vi "HEX-String Languages to Unicode Array.vi"(11 "Config in":T1) -> (3 "Config out":T1)   [LabVIEW 2019, in "Language Selection.lvlib"]
doc: "- - -\nCopyright (c) 2026, Merecs Engineering GmbH"
uses:
  Language Selection.lvlib
  TypeDefs/Cluster Language Configuration.ctl
  Cluster Settings Data.ctl
  TypeDefs/Cluster Language.ctl
  TypeDefs/Cluster PropertyTranslation.ctl
  TypeDefs/Enum Property Type.ctl
  <vilib>/addons/Tools/Unicode/_subVIs/Convert UTF-16LE to ASCII (Scalar).vi
  <vilib>/addons/Tools/Unicode/UI Unicode Tools.lvlib
panel:
  # "Connector Pane"
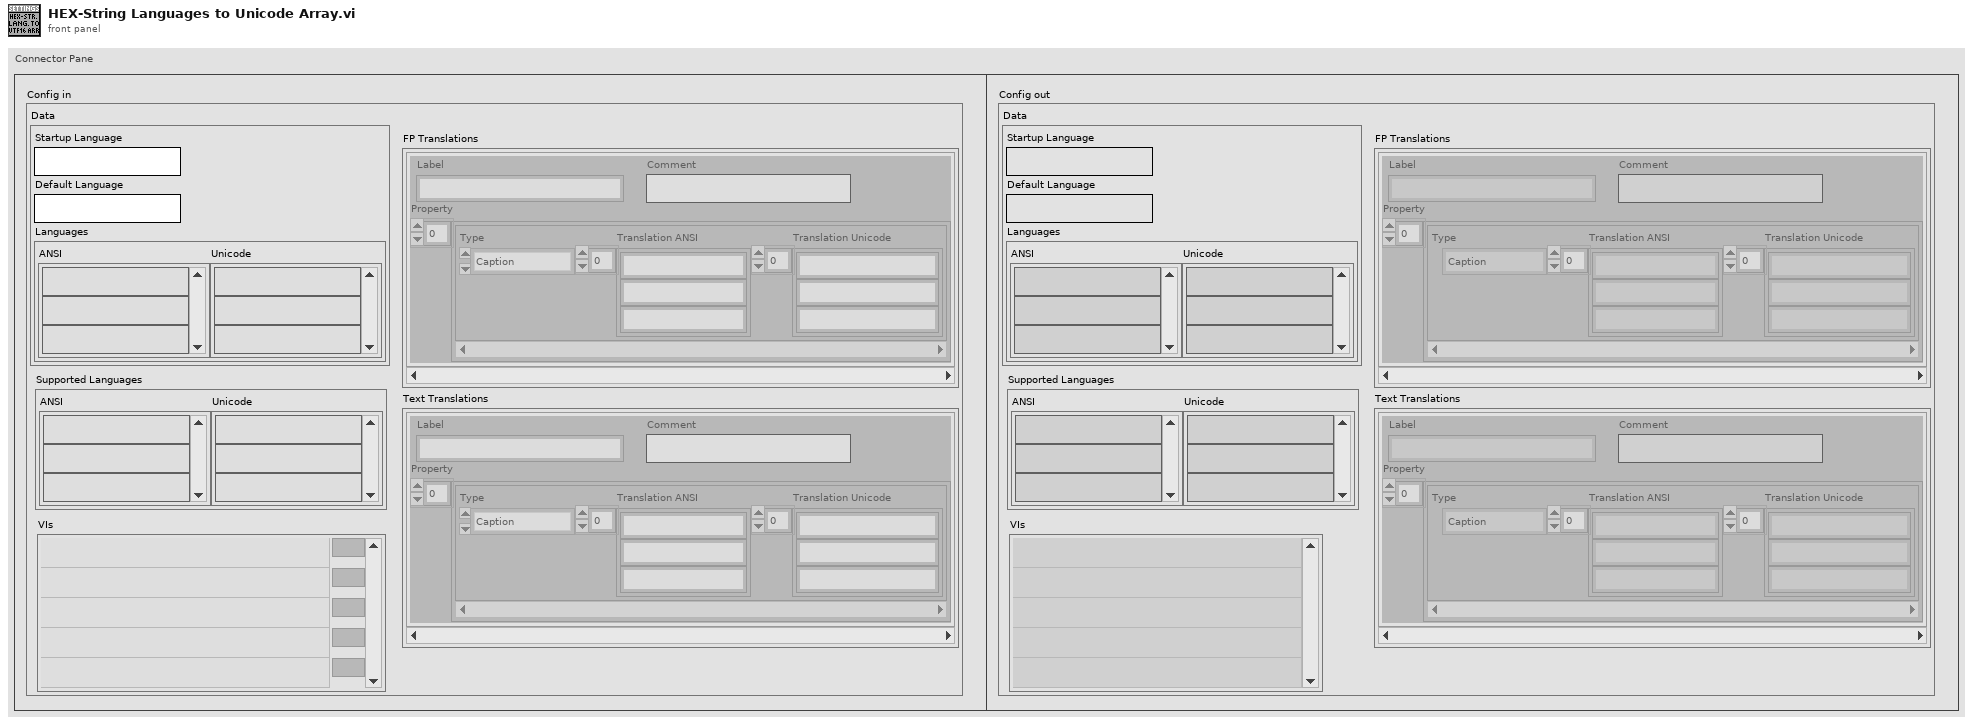
[diagram p1: front panel]
types:
  T1 = typedef "Language Selection.lvlib/Cluster Language Configuration.ctl" = cluster{"Data":T2, "Supported Languages":cluster{"ANSI":string[], "Unicode":string[]}, "VIs":path[], "FP Translations":T3[], "Text Translations":T3[]}
  T2 = typedef "Language Selection.lvlib/Cluster Settings Data.ctl" = cluster{"Startup Language":string, "Default Language":string, "Languages":cluster{"ANSI":string[], "Unicode":string[]}}
  T3 = typedef "Language Selection.lvlib/Cluster Language.ctl" = cluster{"Label":string, "Comment":string, "Property":T4[]}
  T4 = typedef "Language Selection.lvlib/Cluster PropertyTranslation.ctl" = cluster{"Type":T5, "Translation ANSI":string[], "Translation Unicode":string[]}
  T5 = typedef "Language Selection.lvlib/Enum Property Type.ctl" = enum16{"NA", "Caption", "String Value", "Boolean Text", "Ring Strings", "1D Array Elements", "2D Array Elements", "(MC)Listbox Header", "(MC)Listbox Items", "Tab Pages Names", "X & Y GraphChart", "Plot Names", "Table Headers", "Table Items", "TipStrip", "Combobox Strings", "Cursor Name", "Tree Col Headers"}
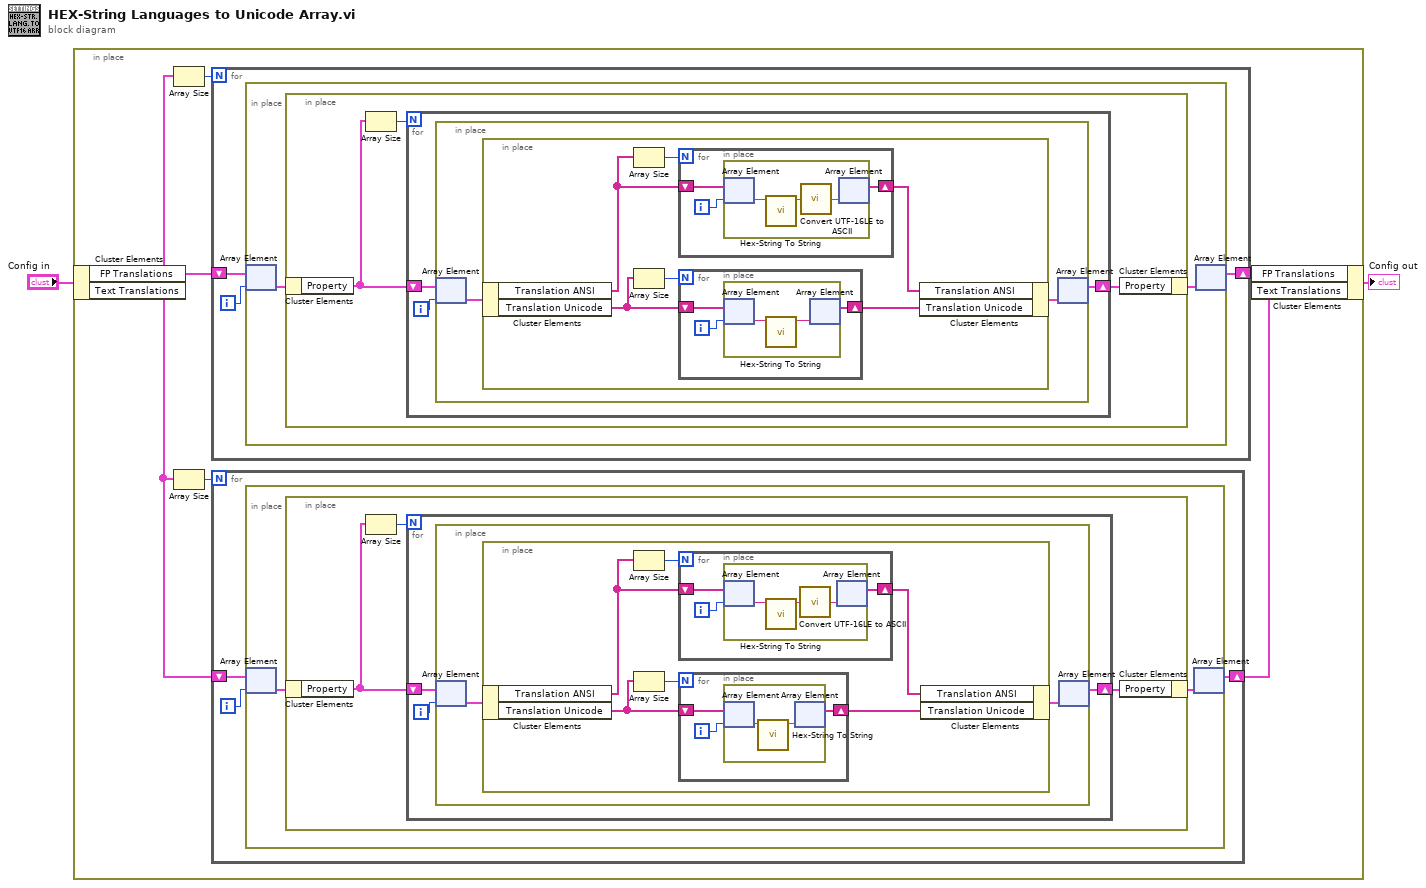
[diagram p0: block diagram]
diagram:
  n1 = in-place {
    n2 = in-place-cluster #1("Config in") -> ("FP Translations"=w7:T3[], "Text Translations"=w4:T3[])
    n3 = Array Size(array=w7) -> (size(s)=w8:i32)
    n4 = Array Size(array=w4) -> (size(s)=w5:i32)
    n5 = for {
      N: w8 -> [_]
      shift-right: [w40] -> w6
      shift-left: w7 -> [w41]
      i -> [w39]
      n6 = in-place {
        n7 = in-place-array #2(w41, w39) -> (w43:T3)
        n8 = in-place {
          n9 = in-place-cluster #3(w43) -> ("Property"=w45:T4[])
          n10 = Array Size(array=w45) -> (size(s)=w46:i32)
          n11 = for {
            N: w46 -> [_]
            shift-right: [w47] -> w44
            shift-left: w45 -> [w49]
            i -> [w48]
            n12 = in-place {
              n13 = in-place-array #4(w49, w48) -> (w51:T4)
              n14 = in-place {
                n15 = in-place-cluster #5(w51) -> ("Translation ANSI"=w53:string[], "Translation Unicode"=w57:string[])
                n16 = Array Size(array=w53) -> (size(s)=w54:i32)
                n17 = Array Size(array=w57) -> (size(s)=w56:i32)
                n18 = for {
                  N: w54 -> [_]
                  shift-right: [w58] -> w52
                  shift-left: w53 -> [w60]
                  i -> [w59]
                  n19 = in-place {
                    n20 = in-place-array #6(w60, w59) -> (w63:string)
                    n21 = call "Hex-String To String.vi"("HEX-String"=w63) -> ("string"=w62:string)  [unwired: 10 in]
                    n22 = call-poly <vilib>:"Convert UTF-16LE to ASCII.vi"("Unicode"=w62) -> ("ASCII"=w61:string)  [unwired: 4 in]
                    n23 = in-place-array #6(w61) -> (w58:string[])  [unwired: 1 out]
                  }
                }
                n24 = for {
                  N: w56 -> [_]
                  shift-right: [w64] -> w55
                  shift-left: w57 -> [w66]
                  i -> [w65]
                  n25 = in-place {
                    n26 = in-place-array #7(w66, w65) -> (w68:string)
                    n27 = call "Hex-String To String.vi"("HEX-String"=w68) -> ("string"=w67:string)  [unwired: 10 in]
                    n28 = in-place-array #7(w67) -> (w64:string[])  [unwired: 1 out]
                  }
                }
                n29 = in-place-cluster #5("Translation ANSI"=w52, "Translation Unicode"=w55) -> (w50:T4)
              }
              n30 = in-place-array #4(w50) -> (w47:T4[])  [unwired: 1 out]
            }
          }
          n31 = in-place-cluster #3("Property"=w44) -> (w42:T3)
        }
        n32 = in-place-array #2(w42) -> (w40:T3[])  [unwired: 1 out]
      }
    }
    n33 = for {
      N: w5 -> [_]
      shift-right: [w10] -> w3
      shift-left: w4 -> [w11]
      i -> [w9]
      n34 = in-place {
        n35 = in-place-array #8(w11, w9) -> (w13:T3)
        n36 = in-place {
          n37 = in-place-cluster #9(w13) -> ("Property"=w15:T4[])
          n38 = Array Size(array=w15) -> (size(s)=w16:i32)
          n39 = for {
            N: w16 -> [_]
            shift-right: [w17] -> w14
            shift-left: w15 -> [w19]
            i -> [w18]
            n40 = in-place {
              n41 = in-place-array #10(w19, w18) -> (w21:T4)
              n42 = in-place {
                n43 = in-place-cluster #11(w21) -> ("Translation ANSI"=w23:string[], "Translation Unicode"=w27:string[])
                n44 = Array Size(array=w23) -> (size(s)=w24:i32)
                n45 = Array Size(array=w27) -> (size(s)=w26:i32)
                n46 = for {
                  N: w24 -> [_]
                  shift-right: [w28] -> w22
                  shift-left: w23 -> [w30]
                  i -> [w29]
                  n47 = in-place {
                    n48 = in-place-array #12(w30, w29) -> (w33:string)
                    n49 = call "Hex-String To String.vi"("HEX-String"=w33) -> ("string"=w32:string)  [unwired: 10 in]
                    n50 = call-poly <vilib>:"Convert UTF-16LE to ASCII.vi"("Unicode"=w32) -> ("ASCII"=w31:string)  [unwired: 4 in]
                    n51 = in-place-array #12(w31) -> (w28:string[])  [unwired: 1 out]
                  }
                }
                n52 = for {
                  N: w26 -> [_]
                  shift-right: [w34] -> w25
                  shift-left: w27 -> [w36]
                  i -> [w35]
                  n53 = in-place {
                    n54 = in-place-array #13(w36, w35) -> (w38:string)
                    n55 = call "Hex-String To String.vi"("HEX-String"=w38) -> ("string"=w37:string)  [unwired: 10 in]
                    n56 = in-place-array #13(w37) -> (w34:string[])  [unwired: 1 out]
                  }
                }
                n57 = in-place-cluster #11("Translation ANSI"=w22, "Translation Unicode"=w25) -> (w20:T4)
              }
              n58 = in-place-array #10(w20) -> (w17:T4[])  [unwired: 1 out]
            }
          }
          n59 = in-place-cluster #9("Property"=w14) -> (w12:T3)
        }
        n60 = in-place-array #8(w12) -> (w10:T3[])  [unwired: 1 out]
      }
    }
    n61 = in-place-cluster #1("FP Translations"=w6, "Text Translations"=w3) -> (→"Config out":T1)
  }
